vi "Initialize.vi"(8 "error in (no error)":errorcluster) -> (0 "error out":errorcluster)   [LabVIEW 2020, in "wiringPi.lvlib"]
doc: "<b>_______________________________________________________________</b>\n** Author: Juan José Villacorta\n** LabVIEW wrapper for C library <b> wiringPi </b>,\n** https://github.com/WiringPi/WiringPi\n<b>_______________________________________________________________</b>\n\n\n/*\n * wiringPiSetupGpio:\n * Must be called once at the start of your program execution.\n *\n * GPIO setup: Initialises the system into GPIO Pin mode and uses the\n * memory mapped hardware directly.\n *********************************************************************************\n */"
uses:
  wiringPi.lvlib
  <vilib>/ErrorRing/Error Ring.xnode
  <vilib>/Utility/error.llb/Error Cluster From Error Code.vi
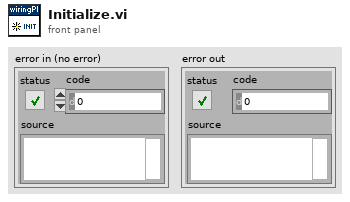
[diagram p1: front panel]
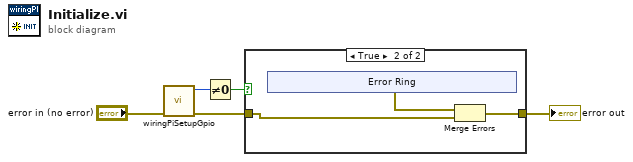
[diagram p0: block diagram]
diagram:
  n1 = call "wiringPiSetupGpio.vi"("error in (no error)"="error in (no error)") -> ("error out"=w2:errorcluster, "status"=w4:i32)  [unwired: 9 in]
  n2 = Not Equal To 0?(x=w4) -> (x != 0?=w3:bool)
  n3 = case shown="True" w3 {
    tunnel: w2 -> [w6 w7]
    tunnel: [w6 w9] -> w1
    frame False {
    }
    frame True {
      n4 = xnode "Error Ring"() -> ("error out"=w8:errorcluster)
      n5 = Merge Errors(w8, w7) -> (w9:errorcluster)
    }
  }
  "error out" <- w1
